vi "Table_UI.vi"(5 "Sort Type":enum16{"numerical", "hex", "string"}(ring), 6 "Table Control":refnum<vi>, 7 "Sort by":u16(ring) items=["Packet_Number", "Timestamp", "Source", "Destination", "Protocol", "Length", "Data"], 8 "error in":errorcluster, 9 "Filter String":string="Protocol == UDP AND Length > 0.7 OR Source == 192.168.1.1", 10 "Headers":string[](array[string])=["Packet Number", "Timestamp", "Source", "Destination", "Protocol", "Length", "Data"], 11 "Unsorted Data":string[][](array[string])) -> (0 "Error Out":errorcluster, 3 "Table Control":string[][](table))   [LabVIEW 2025, in "Automotive Ethernet Bus Monitor UI.lvlib" / "Table_Filtering.lvlib"]
uses:
  Table_Filtering.lvlib
  <vilib>/Utility/miscctls.llb/LVBoundsTypeDef.ctl
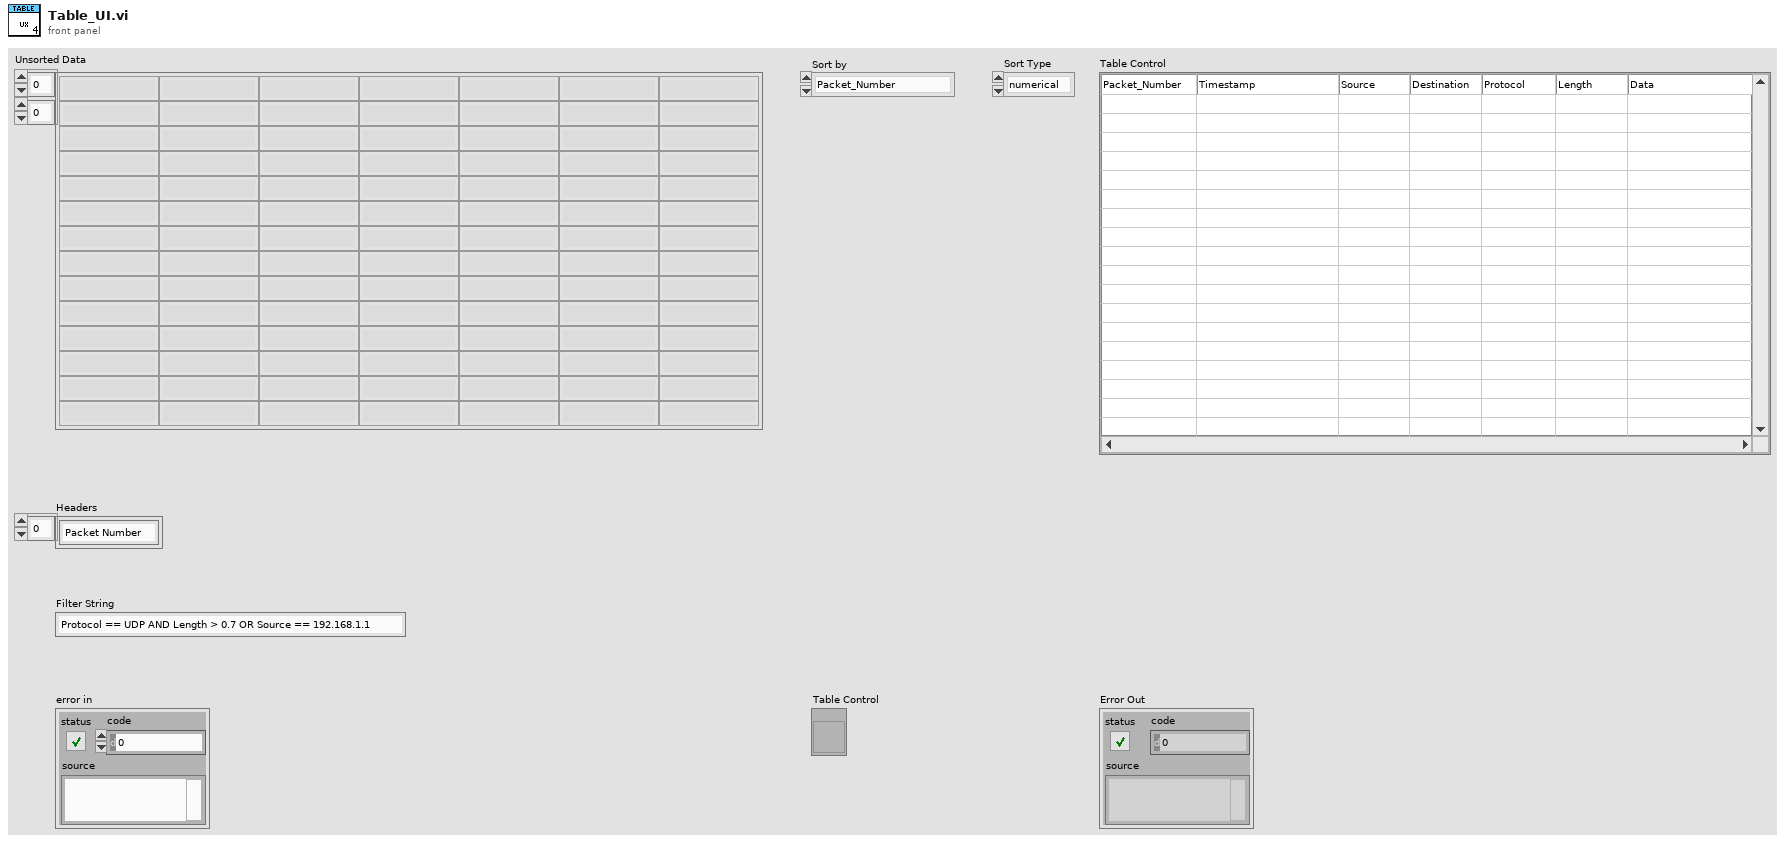
[diagram p1: front panel]
types:
  T1 = typedef "LVBoundsTypeDef.ctl" = cluster{"Width":u32, "Height":u32}
  T2 = cluster{"FIELD":string, "OPERATOR":string, "VALUE":string}[]
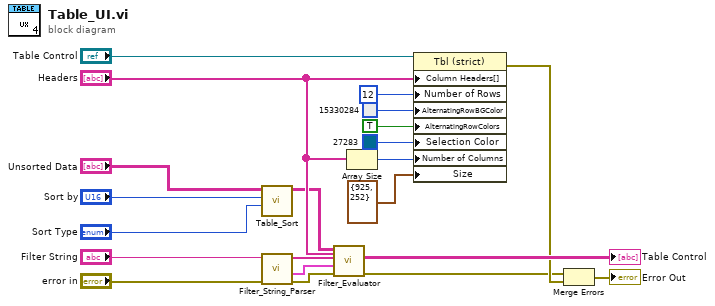
[diagram p0: block diagram]
diagram:
  n1 = call "Table_Sort.vi"("Sort Type"="Sort Type", "Sort by"="Sort by", "Unsorted Data"="Unsorted Data") -> ("Sorted data"=w11:string[][])  [unwired: 8 in]
  n2 = call "Filter_String_Parser.vi"("error in"="error in", "Filter String"="Filter String") -> ("error constant"=w13:errorcluster, "Comparators"=w20:T2, "Boolean Connectors"=w19:string[])  [unwired: 7 in]
  n3 = call "Filter_Evaluator.vi"("Headers"="Headers", "Error"=w13, "Comparators"=w20, "Boolean Connectors"=w19, "Prefiltered Data"=w11) -> ("Error Out"=w5:errorcluster, "Filtered Array"=→"Table Control":string[][])  [unwired: 4 in, 1 out]
  n4 = Array Size(array="Headers") -> (size(s)=w17:i32)
  n5 = property on="Property Node" class="Tbl (strict)"(reference="Table Control", "Column Headers[]"="Headers", "Number of Rows"=12 ("y"), "AlternatingRowBGColor"=u32 15330284 ("Alternate Row Background Color"), "AlternatingRowColors"=TRUE ("Alternating Row Colors"), "Selection Color"=u32 27283, "Number of Columns"=w17, "Size"=T1 {"Width"=925, "Height"=252}) -> (error out=w6:errorcluster)  [unwired: 1 in, 1 out]
  n6 = Merge Errors(w5, w6) -> (→"Error Out":errorcluster)
